vi "Query Antenna Pol.vi"(8 "error in (no error)":errorcluster, 11 "CO3000 in":refnum<class "CO3000.lvclass">) -> (0 "error out":errorcluster, 2 "Antenna Pol":string, 3 "CO3000 out":refnum<class "CO3000.lvclass">)   [LabVIEW 2023, in "Turn Table and Mast.lvlib" / "CO3000.lvclass"]
uses:
  CO3000.lvclass
  CO3000.lvclass/CO3000.ctl
  <vilib>/Utility/error.llb/Error Cluster From Error Code.vi
  <vilib>/ErrorRing/Error Ring.xnode
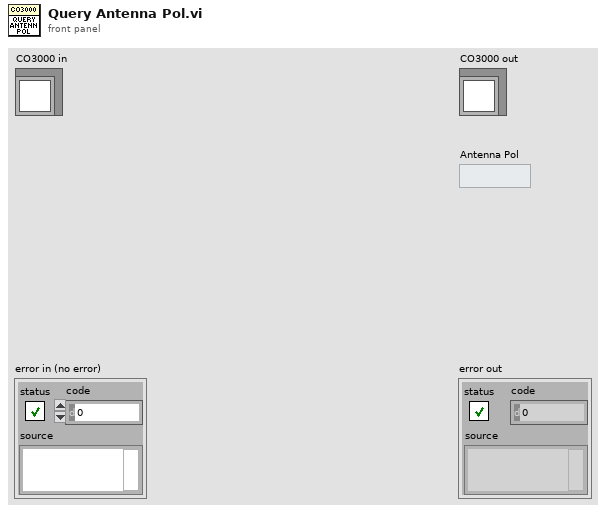
[diagram p1: front panel]
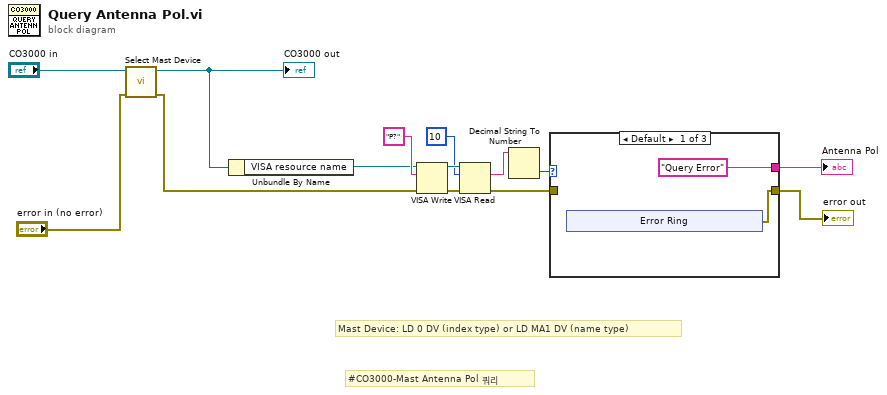
[diagram p0: block diagram]
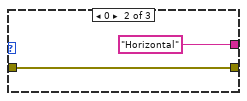
[diagram p2: hidden frame]
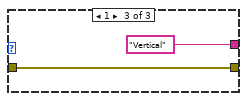
[diagram p3: hidden frame]
diagram:
  # "#CO3000-Mast Antenna Pol 쿼리"
  # "Mast Device: LD 0 DV (index type) or LD MA1 DV (name type)"
  n1 = call "Select Mast Device.vi"("error in (no error)"="error in (no error)", "CO3000 in"="CO3000 in") -> ("error out"=w1:errorcluster, "CO3000 out"=w4:refnum<class "CO3000.lvclass">)  [unwired: 8 in]
  "CO3000 out" <- w4
  n2 = Unbundle By Name(w4) -> ("VISA resource name"=w2:refnum<visa-resource-name>)
  n3 = VISA Write(VISA resource name=w2, write buffer="P?" ("버퍼 쓰기"), error in (no error)=w1) -> (VISA resource name out=w12:refnum<visa-resource-name>, error out=w13:errorcluster)  [unwired: 1 out]
  n4 = VISA Read(VISA resource name=w12, byte count=u32 10 ("바이트 카운트"), error in (no error)=w13) -> (read buffer=w10:string, error out=w8:errorcluster)  [unwired: 2 out]
  n5 = Decimal String To Number(string=w10) -> (number=w9:i32)  [unwired: 2 in, 1 out]
  n6 = case shown="Default" w9 {
    tunnel: w8 -> [_ w23 w25]
    tunnel: [w15 w23 w25] -> w6
    tunnel: ["Query Error" "Horizontal" "Vertical"] -> w7
    frame Default {
      n7 = xnode "Error Ring"() -> ("error out"=w15:errorcluster)
    }
    frame 0 {
    }
    frame 1 {
    }
  }
  "error out" <- w6
  "Antenna Pol" <- w7
